vi "Destroy.vi"(8 "error in (no error)":errorcluster, 11 "Icoryx_PCAP in":refnum<class "CIF_Iceoryx_PCAP_Universal.lvclass">) -> (0 "error out":errorcluster, 3 "Icoryx_PCAP out":refnum<class "CIF_Iceoryx_PCAP_Universal.lvclass">)   [LabVIEW 2021, in "CIF_Iceoryx_PCAP_Universal.lvclass"]
uses:
  CIF_Iceoryx_PCAP_Universal.lvclass
  D:/dev/Packages/CIF_Channels_Core/src/CIFChannels/CIFChannels.lvclass
  CIFChannels/CIFChannels.lvclass/CIFChannels.ctl
  ChannelCommon/typedef/Channel State.ctl
  CIF_Iceoryx_PCAP_Universal.lvclass/CIF_Iceoryx_PCAP_Universal.ctl
  CIFChannels/Accessors/Read Direction.vi
  CIFChannels/Accessors/Write Subscriber Count.vi
  CIFChannels/Accessors/Write Channel State.vi
  CIFChannels/Accessors/Write Publisher Name.vi
  ChannelCommon/ChannelCommon.lvlib
  <vilib>/CIF Foundation/CIF Iceoryx/Iceoryx.lvlib
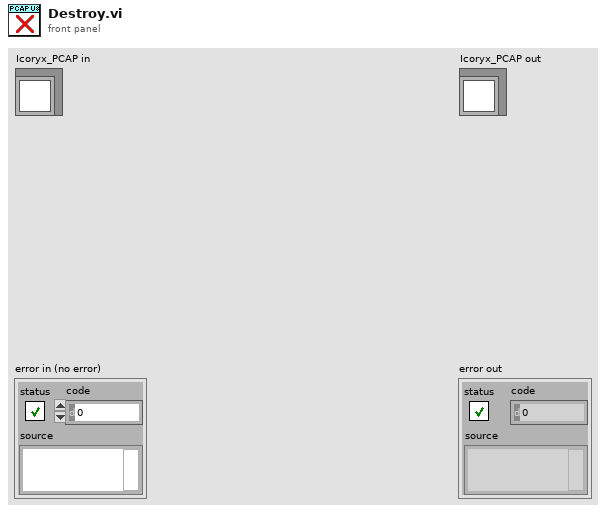
[diagram p1: front panel]
types:
  T1 = typedef "ChannelCommon.lvlib/Channel State.ctl" = enum8{"Creating", "Disconnected", "Connecting", "Connected", "Destroyed"}
  T2 = typedef "ChannelCommon.lvlib/Direction.ctl" = enum8{"Publisher", "Subscriber"}
  T3 = typedef "Iceoryx.lvlib/CIF Publisher Refnum.ctl" = cluster{"refnum":u64, "CIF Pub":enum8{"cifpub"}}
  T4 = typedef "Iceoryx.lvlib/CIF Subscriber Refnum.ctl" = cluster{"refnum":u64, "CIF Sub":enum8{"cifsub"}}
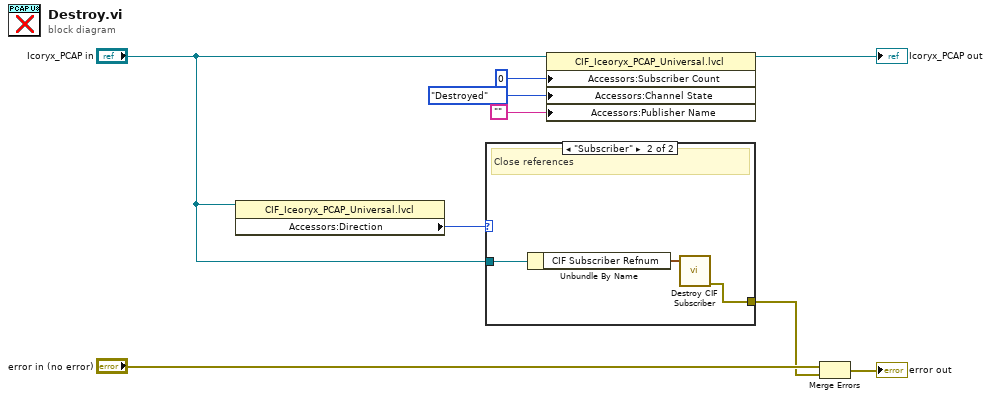
[diagram p0: block diagram]
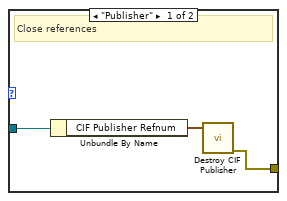
[diagram p2: hidden frame]
diagram:
  n1 = property class="CIF_Iceoryx_PCAP_Universal.lvcl"(reference="Icoryx_PCAP in") -> ("Accessors:Direction"=w6:T2)  [unwired: 1 in, 2 out]
  n2 = case shown="\"Subscriber\"" w6 {
    tunnel: [w12 w15] -> w5
    tunnel: "Icoryx_PCAP in" -> [w11 w14]
    frame "Publisher" {
      # "Close references"
      n3 = Unbundle By Name(w11) -> ("CIF Publisher Refnum"=w10:T3)
      n4 = call <vilib>:"Destroy CIF Publisher.vi"("Publisher Reference"=w10) -> ("error out"=w12:errorcluster)  [unwired: 10 in]
    }
    frame "Subscriber" {
      # "Close references"
      n5 = Unbundle By Name(w14) -> ("CIF Subscriber Refnum"=w13:T4)
      n6 = call <vilib>:"Destroy CIF Subscriber.vi"("Subscriber Reference"=w13) -> ("error out"=w15:errorcluster)  [unwired: 10 in]
    }
  }
  n7 = property class="CIF_Iceoryx_PCAP_Universal.lvcl"(reference="Icoryx_PCAP in", "Accessors:Subscriber Count"=u32 0 ("Subscriber Count"), "Accessors:Channel State"=Channel_State."Destroyed" ("Channel State"), "Accessors:Publisher Name"="") -> (reference out=→"Icoryx_PCAP out":refnum<class "CIF_Iceoryx_PCAP_Universal.lvclass">)  [unwired: 1 in, 1 out]
  n8 = Merge Errors("error in (no error)", w5) -> (→"error out":errorcluster)
